vi "FuncVI_Sub - File - convert slashes within file path.vi"(0 "str: path":string) -> (2 "str: path out":string, 3 "path out":path)   [LabVIEW 2021]
doc: "::: CalcExpress Toolkit :::\nCopyright (c) 2000-2026 Konstantin Shifershteyn. All rights reserved."
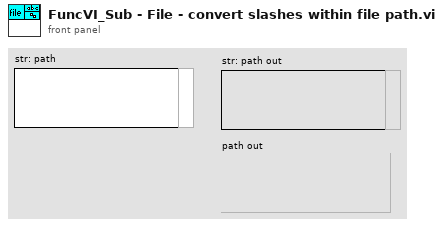
[diagram p1: front panel]
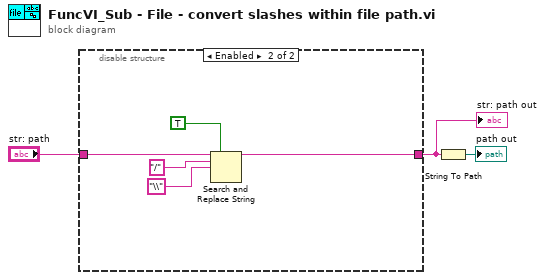
[diagram p0: block diagram]
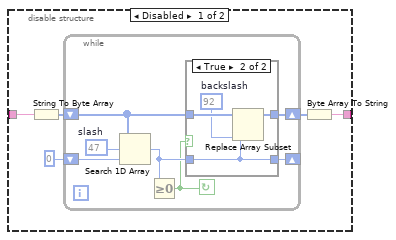
[diagram p2: hidden frame]
diagram:
  n1 = disable-structure shown="Enabled" {
    disable-tunnel: [w5 w24] -> w2
    disable-tunnel: "str: path" -> [w4 w25]
    frame Disabled {
      n2 = String To Byte Array(string=w4) -> (unsigned byte array=w8:u8[])
      n3 = while {
        shift-left: 0 -> [w14]
        shift-right: [w13] -> _
        shift-left: w8 -> [w11]
        shift-right: [w10] -> w6
        stop <- w9 continue-if-true
        w15 = u8 47  # slash
        n4 = Search 1D Array(1D array=w11, element=w15, start index (0)=w14) -> (index of element=w12:i32)
        n5 = Greater Or Equal To 0?(x=w12) -> (x >= 0?=w9:bool)
        n6 = case shown="True" w9 {
          tunnel: [w16 w21] -> w13
          tunnel: w12 -> [w16 w21]
          tunnel: w11 -> [w17 w20]
          tunnel: [w17 w19] -> w10
          frame False {
          }
          frame True {
            w18 = u8 92  # backslash
            n7 = Replace Array Subset(array=w20, new element=w18, index=w21) -> (w19:u8[])
          }
        }
      }
      n8 = Byte Array To String(unsigned byte array=w6) -> (string=w5:string)
    }
    frame Enabled {
      n9 = Search and Replace String(replace all?=TRUE, input string=w25, search string="/", replace string="\\" ("replace string (\"\")")) -> (result string=w24:string)  [unwired: 4 in, 3 out]
    }
  }
  "str: path out" <- w2
  n10 = String To Path(string=w2) -> (path=→"path out":path)
